vi "control_aeropendulo_LabVIEW2020.vi"() -> ()   [LabVIEW 2020]
panel:
  in  "Corte (grados)":dbl=45.0
  out "Estado swing up":dbl=2.0
  in  "Tope (grados)":dbl=-69.7
  in  "MODO DE ARRANQUE":dbl(ring) items=["Vertical: sostener a mano y soltar", "Swing up desde tope IZQUIERDO", "Swing up desde tope DERECHO"]
  in  "V pulsos":dbl
  in  "V cerca de 0":dbl
  in  "Vr reposo":dbl
  in  "Kv actuador":dbl=0.6
  in  "Invertir sentido 2":bool=TRUE caption="PWM invertido"
  out "Grafica del error y banda de 2 grados":cluster{"errdeg":dbl, dbl, dbl}(graph)={"errdeg"=70.16, 2.0, -2.0}
  out "Grafica angulo vs referencia y limites 2 grados":T1(graph)={"thdeg"=-70.16, "Referencia (grados)"=0.0, 2.0, -2.0}
  out "Angulo de la varilla (grados)":dbl(knob)=-70.16 scale=-75.0..75.0
  out "Error (grados)":dbl=70.16
  out "Motor activo (0 apagado, 1 o 2)":dbl
  out "Voltaje a la AO (V)":dbl
  out "Salida del control u":dbl=1.1396014156972711
  in  "STOP":bool
  in  "Invertir sentido":bool=TRUE
  in  "Habilitar motores":bool=TRUE
  in  "Modo automatico":bool=TRUE
  in  "Tarar (cero aqui)":bool
  in  "Vmax AO (V)":dbl=5.0
  in  "Angulo limite (grados)":dbl=90.0
  in  "Voff arranque motor (V)":dbl=0.2
  in  "Voltaje manual (V AO)":dbl=0.1
  in  "Motor manual (1 o 2)":dbl=1.0
  in  "Kd":dbl(knob)=0.9 scale=0.0..2.0
  in  "Ki":dbl(knob)=0.4 scale=0.0..2.0
  in  "Kp":dbl(knob)=2.0 scale=0.0..10.0
  in  "Referencia (grados)":dbl(knob) scale=-10.0..10.0
  # "MODO DE ARRANQUE"
  # "CÓMO USAR\n1. Elegir el MODO DE ARRANQUE:\n   - Vertical: sostener la varilla derecha, Run y soltar.\n   - Swing up: varilla quieta en ESE tope, Run (no tocarla).\n2. Habilitar motores y Modo automático en ON (verde).\n3. Para apagar: Habilitar en OFF y luego STOP.\nEstado swing up: 0 sube, 1 planea, 2 sostiene,\n3 no despegó (revisar el lado del tope)."
  # "Invertir sentido"
  # "PWM invertido"
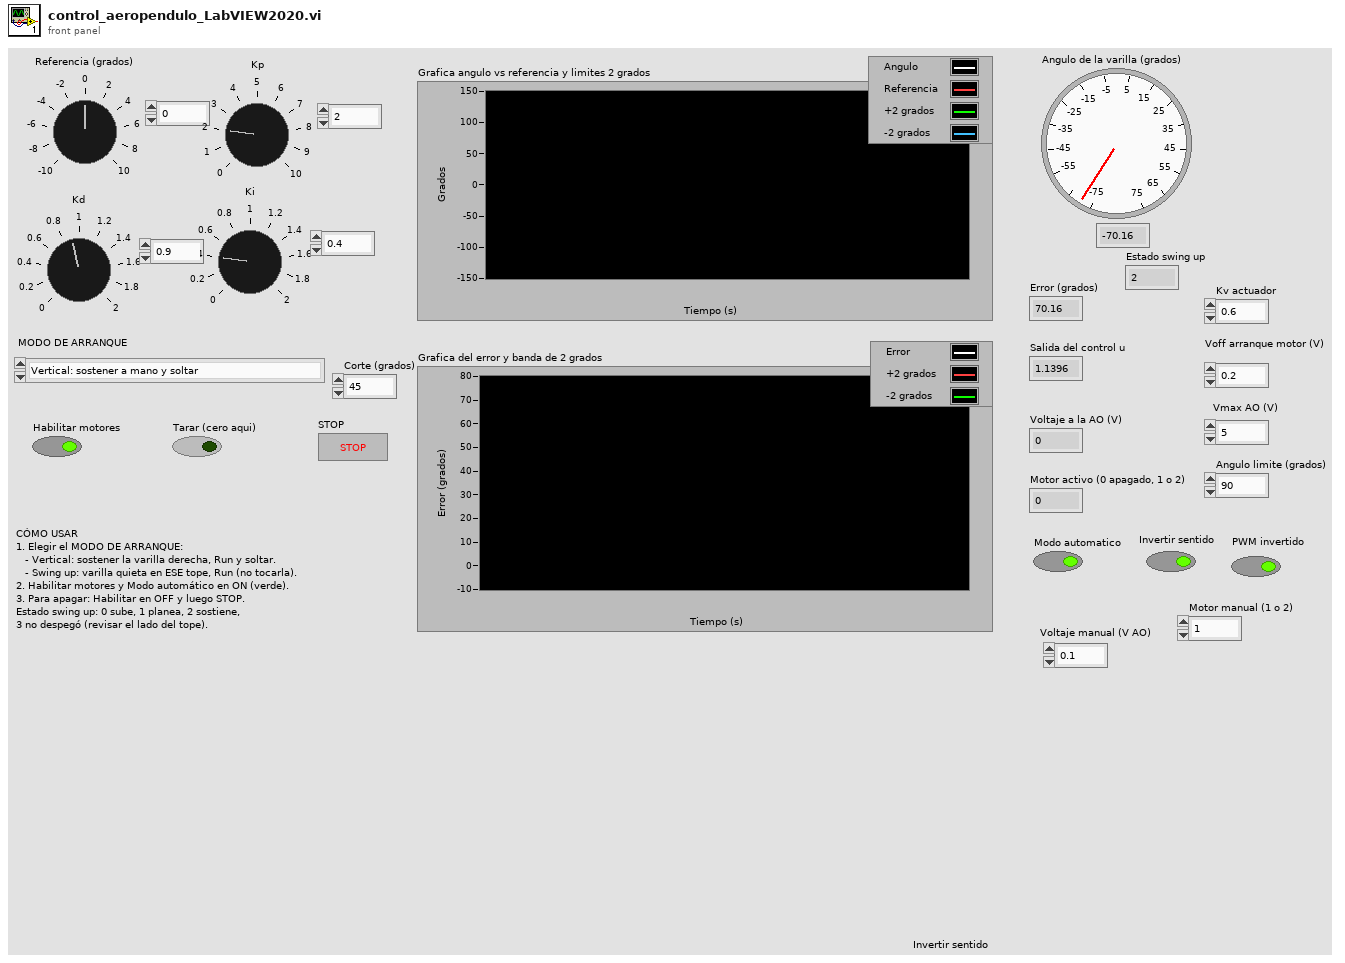
[diagram p1: front panel]
types:
  T1 = cluster{"thdeg":dbl, "Referencia (grados)":dbl, dbl, dbl}
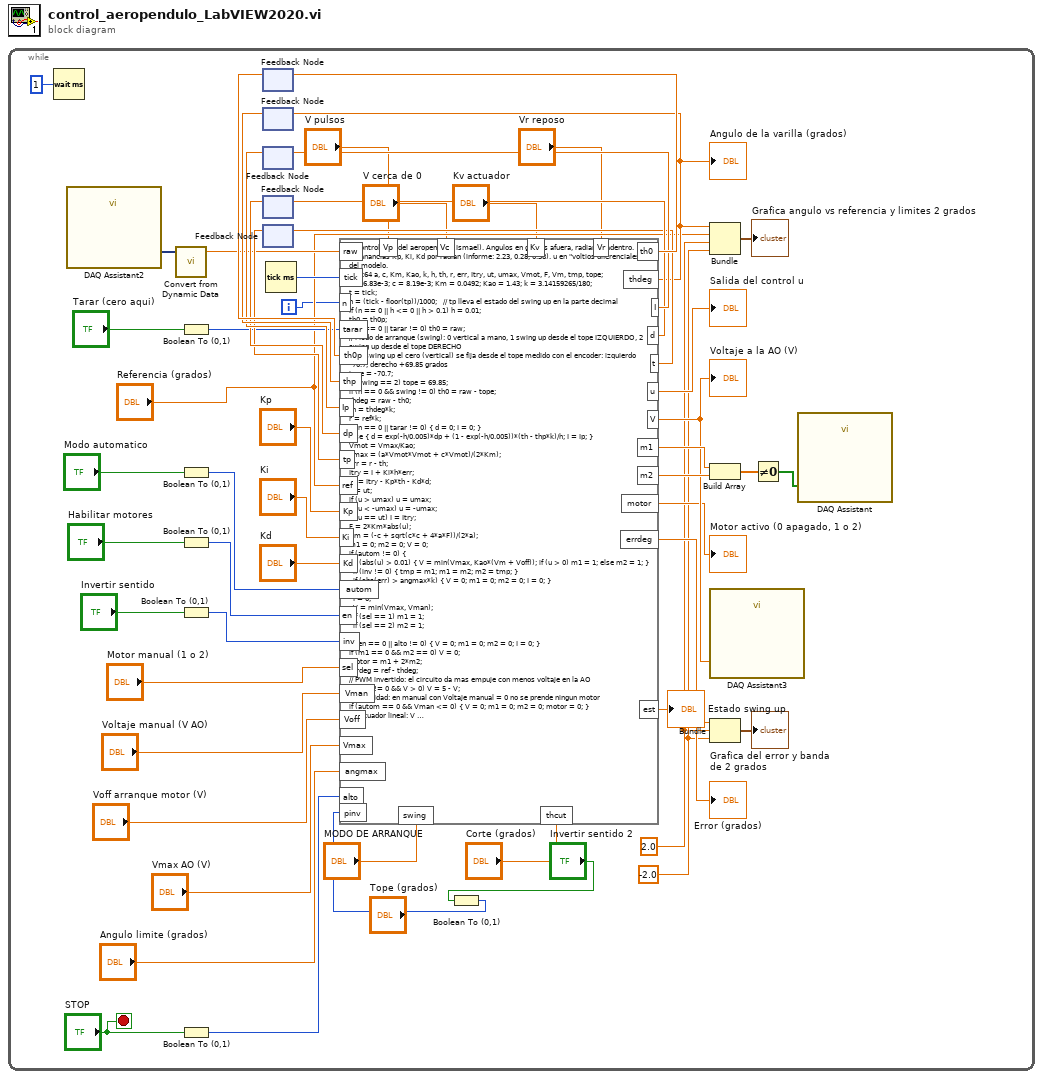
[diagram p0: block diagram]
diagram:
  n1 = while {
    i -> [w11]
    stop <- "STOP" stop-if-true
    w14 = -2.0
    w8 = 2.0
    n2 = Wait (ms)(milliseconds to wait=u32 1) -> ()  [unwired: 1 out]
    n3 = call "DAQ Assistant2"() -> ("data"=w25:dynamicdata)  [unwired: 16 in, 3 out]
    n4 = call "Convert from Dynamic Data"("Dynamic Data Type"=w25) -> ("Scalar"=w24:dbl)  [unwired: 3 in]
    n5 = Boolean To (0,1)(Boolean="Tarar (cero aqui)") -> (0, 1=w36:i16)
    n6 = Boolean To (0,1)(Boolean="Modo automatico") -> (0, 1=w35:i16)
    n7 = Boolean To (0,1)(Boolean="Habilitar motores") -> (0, 1=w34:i16)
    n8 = Boolean To (0,1)(Boolean="Invertir sentido") -> (0, 1=w33:i16)
    n9 = Boolean To (0,1)(Boolean="STOP") -> (0, 1=w21:i16)
    n10 = feedback #1() -> (w54:dbl)  [unwired: 1 in]
    n11 = feedback #2() -> (w53:dbl)  [unwired: 1 in]
    n12 = feedback #3() -> (w51:dbl)  [unwired: 1 in]
    n13 = feedback #4() -> (w49:dbl)  [unwired: 1 in]
    n14 = feedback #5() -> (w47:dbl)  [unwired: 1 in]
    n15 = Tick Count (ms)() -> (millisecond timer value=w46:u32)
    n16 = Boolean To (0,1)(Boolean="Invertir sentido 2") -> (0, 1=w9:i16)
    n17 = formula code="// Control I-PD del aeropendulo (Ismael). Angulos en grados afuera, radianes adentro.\n// Ganancias Kp, Ki, Kd por radian (informe: 2.23, 0.28, 0.38). u en \"voltios diferenciales\" del modelo.\nfloat64 a, c, Km, Kao, k, h, th, r, err, Itry, ut, umax, Vmot, F, Vm, tmp, tope;\na = 6.83e-3; c = 8.19e-3; Km = 0.0492; Kao = 1.43; k = 3.14159265/180;\nt = tick;\nh = (tick - floor(tp))/1000;   // tp lleva el estado del swing up en la parte decimal\nif (n == 0 || h <= 0 || h > 0.1) h = 0.01;\nth0 = th0p;\nif (n == 0 || tarar != 0) th0 = raw;\n// Modo de arranque (swing): 0 vertical a mano, 1 swing up desde el tope IZQUIERDO, 2 swing up desde el tope DERECHO\n// En swing up el cero (vertical) se fija desde el tope medido con el encoder: izquierdo -70.7, derecho +69.85 grados\ntope = -70.7;\nif (swing == 2) tope = 69.85;\nif (n == 0 && swing != 0) th0 = raw - tope;\nthdeg = raw - th0;\nth = thdeg*k;\nr = ref*k;\nif (n == 0 || tarar != 0) { d = 0; I = 0; }\nelse { d = exp(-h/0.005)*dp + (1 - exp(-h/0.005))*(th - thp*k)/h; I = Ip; }\nVmot = Vmax/Kao;\numax = (a*Vmot*Vmot + c*Vmot)/(2*Km);\nerr = r - th;\nItry = I + Ki*h*err;\nut = Itry - Kp*th - Kd*d;\nu = ut;\nif (u > umax) u = umax;\nif (u < -umax) u = -umax;\nif (u == ut) I = Itry;\nF = 2*Km*abs(u);\nVm = (-c + sqrt(c*c + 4*a*F))/(2*a);\nm1 = 0; m2 = 0; V = 0;\nif (autom != 0) {\n  if (abs(u) > 0.01) { V = min(Vmax, Kao*(Vm + Voff)); if (u > 0) m1 = 1; else m2 = 1; }\n  if (inv != 0) { tmp = m1; m1 = m2; m2 = tmp; }\n  if (abs(err) > angmax*k) { V = 0; m1 = 0; m2 = 0; I = 0; }\n} else {\n  I = 0;\n  V = min(Vmax, Vman);\n  if (sel == 1) m1 = 1;\n  if (sel == 2) m2 = 1;\n}\nif (en == 0 || alto != 0) { V = 0; m1 = 0; m2 = 0; I = 0; }\nif (m1 == 0 && m2 == 0) V = 0;\nmotor = m1 + 2*m2;\nerrdeg = ref - thdeg;\n// PWM invertido: el circuito da mas empuje con menos voltaje en la AO\nif (pinv != 0 && V > 0) V = 5 - V;\n// Seguridad: en manual con Voltaje manual = 0 no se prende ningun motor\nif (autom == 0 && Vman <= 0) { V = 0; m1 = 0; m2 = 0; motor = 0; }\n// Actuador lineal: V = Voff + Kv*|u| (reemplaza la curva de empuje del informe)\nif (autom != 0 && (m1 != 0 || m2 != 0)) { V = min(Vmax, Voff + Kv*abs(u)); if (pinv != 0) V = 5 - V; }\n// Motores en reposo: si el control pide menos que Vr, se prenden las DOS lineas con Vr (giran suave y se cancelan); Vr = 0 lo desactiva\nif (Vr > 0 && autom != 0 && en != 0 && alto == 0 && abs(err) <= angmax*k && Voff + Kv*abs(u) < Vr) { m1 = 1; m2 = 1; motor = 3; V = Vr; if (pinv != 0) V = 5 - V; }\n// Limite segun el angulo: cerca de 0 grados el voltaje no pasa de Vc y sube en linea recta hasta Vmax a los 20 grados (Vc = 0 lo desactiva)\nif (Vc > 0 && autom != 0 && (m1 + m2) == 1) { V = min(Vc + (Vmax - Vc)*min(1, abs(thdeg)/20), Voff + Kv*abs(u)); if (pinv != 0) V = 5 - V; }\n// Pulsos: si el control pide menos que Vp, el motor se prende solo una fraccion de cada 5 ciclos (unos 50 ms) con la AO al minimo; Vp = 0 lo desactiva\nif (Vp > 0 && autom != 0 && (m1 + m2) == 1 && Voff + Kv*abs(u) < Vp) { V = 0; if (pinv != 0) V = 5; if (n - 5*floor(n/5) >= 5*(Voff + Kv*abs(u))/Vp) { m1 = 0; m2 = 0; motor = 0; V = 0; } }\n// Swing up (swing = 1 o 2): sube desde el tope y la atrapa. est: 0 subir con empuje maximo, 1 planear con motores apagados, 2 sostener con el I-PD,\n// 3 error: no despego del tope en 1.5 s (lado del tope equivocado o motor sin fuerza) -> motores apagados hasta el proximo Run\nest = floor((tp - floor(tp))*10 + 0.5);   // estado del ciclo anterior (guardado en la parte decimal de t)\nif (n == 0) est = 0;\nif (swing == 0) est = 2;\nif (swing != 0 && autom != 0 && en != 0 && alto == 0) {\n  if (est == 0) { if (abs(thdeg) <= thcut) est = 1; else { I = Ip + h; if (I > 1.5 && abs(thdeg) > 55) est = 3; } }\n  else if (est == 1) { if (abs(thdeg) <= 12) { est = 2; I = 0; } else if (thdeg*d > 0 && abs(d) > 0.05) est = 0; }\n  else if (est == 2 && abs(thdeg) > 35) { est = 0; I = 0; }\n  if (est == 0) { m1 = 0; m2 = 0; if (thdeg < 0) m1 = 1; else m2 = 1; if (inv != 0) { tmp = m1; m1 = m2; m2 = tmp; } motor = m1 + 2*m2; V = Vmax; if (pinv != 0) V = 5 - V; }\n  if (est == 1 || est == 3) { V = 0; m1 = 0; m2 = 0; motor = 0; I = 0; }\n}\nt = tick + est/10;"("raw"=w24, "tick"=w46, "tarar"=w36, "th0p"=w54, "thp"=w53, "Ip"=w51, "dp"=w49, "tp"=w47, "ref"="Referencia (grados)", "Kp"="Kp", "Ki"="Ki", "Kd"="Kd", "autom"=w35, "en"=w34, "inv"=w33, "sel"="Motor manual (1 o 2)", "Vman"="Voltaje manual (V AO)", "Voff"="Voff arranque motor (V)", "angmax"="Angulo limite (grados)", "Vmax"="Vmax AO (V)", "alto"=w21, "n"=w11, "pinv"=w9, "Kv"="Kv actuador", "Vr"="Vr reposo", "Vc"="V cerca de 0", "Vp"="V pulsos", "swing"="MODO DE ARRANQUE", "thcut"="Corte (grados)") -> ("errdeg"=w15:dbl, "th0"=w55:dbl, "thdeg"=w18:dbl, "I"=w52:dbl, "d"=w50:dbl, "t"=w48:dbl, "u"=→"Salida del control u":dbl, "V"=w23:dbl, "m1"=w29:dbl, "m2"=w28:dbl, "motor"=→"Motor activo (0 apagado, 1 o 2)":dbl, "est"=→"Estado swing up":dbl)
    "Voltaje a la AO (V)" <- w23
    "Error (grados)" <- w15
    "Angulo de la varilla (grados)" <- w18
    n18 = feedback-in #1(w55) -> ()
    n19 = feedback-in #2(w18) -> ()
    n20 = feedback-in #3(w52) -> ()
    n21 = feedback-in #4(w50) -> ()
    n22 = feedback-in #5(w48) -> ()
    n23 = Bundle("thdeg"=w18, "Referencia (grados)"="Referencia (grados)", w8, w14) -> (→"Grafica angulo vs referencia y limites 2 grados":T1)  [unwired: 1 in]
    n24 = Build Array(w29, w28) -> (w27:dbl[])
    n25 = call "DAQ Assistant3"("data"=w23) -> ()  [unwired: 17 in, 2 out]
    n26 = Bundle("errdeg"=w15, w8, w14) -> (→"Grafica del error y banda de 2 grados":cluster{"errdeg":dbl, dbl, dbl})  [unwired: 1 in]
    n27 = Not Equal To 0?(x=w27) -> (x != 0?=w26:bool[])
    n28 = call "DAQ Assistant"("data"=w26) -> ()  [unwired: 17 in, 2 out]
  }
